vi "Set Data Binding.vi"(7 "DataTable Source":refnum<class "DataTable.lvclass">, 8 "error in (no error)":errorcluster, 11 "DataGridView in":refnum<class "DataGridView.lvclass">) -> (0 "error out":errorcluster, 3 "DataGridView out":refnum<class "DataGridView.lvclass">)   [LabVIEW 2016, in "DataGrid.lvlib" / "DataGridView.lvclass"]
doc: "This is a simple data binding step that connects the dataTable with all the data in it, into the DataGridView for display. The columns get bound and autogenerated by the datagridview for any object types with native support in this step. The next step is to set any custom column types to define specific object types."
uses:
  DataGridView.lvclass
  DataTable/DataTable.lvclass
  DataTable/DataTable.lvclass/DataTable.ctl
  System.Windows.Forms
  DataGridView.lvclass/DataGridView.ctl
  DataTable/Read DataTable.vi
  Properties/Read DataGridView.vi
  System.Data
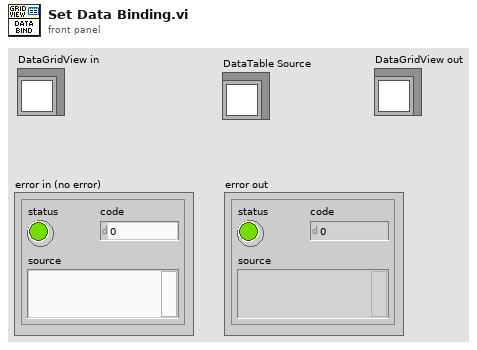
[diagram p1: front panel]
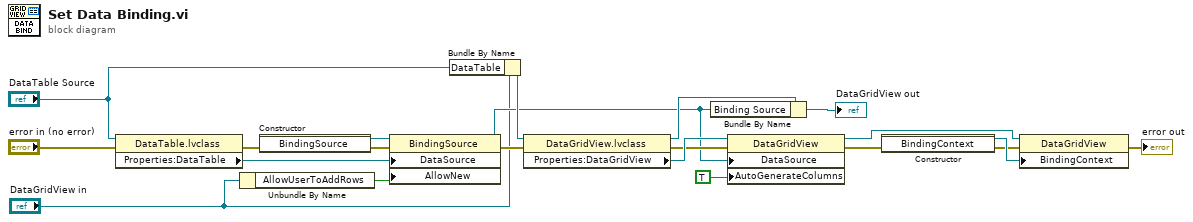
[diagram p0: block diagram]
diagram:
  n1 = property class="DataTable.lvclass"(reference="DataTable Source", error in="error in (no error)") -> (error out=w7:errorcluster, "Properties:DataTable"=w4:refnum<k24>)  [unwired: 1 out]
  n2 = Unbundle By Name("DataGridView in") -> ("AllowUserToAddRows"=w1:bool)
  n3 = constructor class="BindingSource"(error in=w7) -> (reference out=w8:refnum<k24>, error out=w6:errorcluster)  [unwired: 2 in, 1 out]
  n4 = property class="BindingSource"(reference=w8, error in=w6, "DataSource"=w4, "AllowNew"=w1) -> (reference out=w3:refnum<k24>, error out=w5:errorcluster)
  n5 = Bundle By Name(cluster="DataGridView in", "DataTable"="DataTable Source") -> (w12:refnum<class "DataGridView.lvclass">)
  n6 = property class="DataGridView.lvclass"(reference=w12, error in=w5) -> (reference out=w10:refnum<class "DataGridView.lvclass">, error out=w15:errorcluster, "Properties:DataGridView"=w16:refnum<k24>)
  n7 = Bundle By Name(cluster=w10, "Binding Source"=w3) -> (→"DataGridView out":refnum<class "DataGridView.lvclass">)
  n8 = property class="DataGridView"(reference=w16, error in=w15, "DataSource"=w3, "AutoGenerateColumns"=TRUE) -> (reference out=w19:refnum<k24>, error out=w21:errorcluster)
  n9 = constructor class="BindingContext"(error in=w21) -> (reference out=w18:refnum<k24>, error out=w17:errorcluster)  [unwired: 2 in, 1 out]
  n10 = property class="DataGridView"(reference=w19, error in=w17, "BindingContext"=w18) -> (error out=→"error out":errorcluster)  [unwired: 1 out]
